vi "Main Page.vi"(8 "error in (no error)":errorcluster, 11 "Node Ptr":T3 format="%.0x") -> (0 "error out":errorcluster)   [LabVIEW 2025, in "Protection and Counter Addon System Explorer.lvlib"]
uses:
  Protection and Counter Addon System Explorer.lvlib
  <vilib>/NI VeriStand/Custom Device API/Custom Device Item Ref.ctl
  SubModules/Frame-Protection-Support/Source/Shared/Types/Protection Type.ctl
  <vilib>/NI/NI VeriStand Hardware Resource Discovery/_Types/Filter Type.ctl
  Addon Shared/Types/986x.ctl
  Addon Shared/SubVIs/GUID Lookup.vi
  <vilib>/NI VeriStand/Custom Device API/NI VeriStand - Get Item Property.vi
  <vilib>/NI VeriStand/Custom Device API/Get Item Property (Boolean).vi
  <vilib>/NI VeriStand/Custom Device API/Get Item Property (String).vi
  <vilib>/NI VeriStand/Custom Device API/Get Item Property (Dependent File).vi
  <vilib>/NI VeriStand/Custom Device API/Custom Device API.lvlib
  <vilib>/NI/NI VeriStand Hardware Resource Discovery/NIVS Hardware Discovery.lvlib
  Addon Shared/Protection and Counter Addon Shared.lvlib
  SubModules/Frame-Protection-Support/Source/Shared/Protection and Counter Support Shared.lvlib
panel:
  in  "Header":cluster{"Section Name":string}={"Section Name"="Addon Settings"}
  in  "Tab Control":T1(tab)
  in  "FD ISO Mode":u32(ring) items=["ISO", "Non ISO", "ISO Legacy"]
  in  "Description":string
  in  "Name":string
  out "Version":string
  in  "Port":string
  in  "CAN Browse":bool
  out "XNET Database":refnum<k21>
  out "XNET Cluster":refnum<k21>
  out "I/O Mode":u32(ring) items=["CAN 2.0", "CAN FD", "CAN FD+BRS"]
  in  "Baud Rate":u64
  in  "Termination":enum16{"Off", "On"}(ring)
  in  "FD Baud Rate":u64
  in  "Use Legacy":bool
  in  "Loop Priority":i32=100 format="%.0p"
  in  "Enable Bitfile":bool
  in  "Bitfile Path":path
  in  "RIO Device":string
  in  "RIO Browse":bool
  in  "Include All Channels":bool
  in  "Default Protect Type":T2
  in  "Default Max Counter Value":dbl
  in  "SHDocVw.IWebBrowser2":refnum<k7>(container)
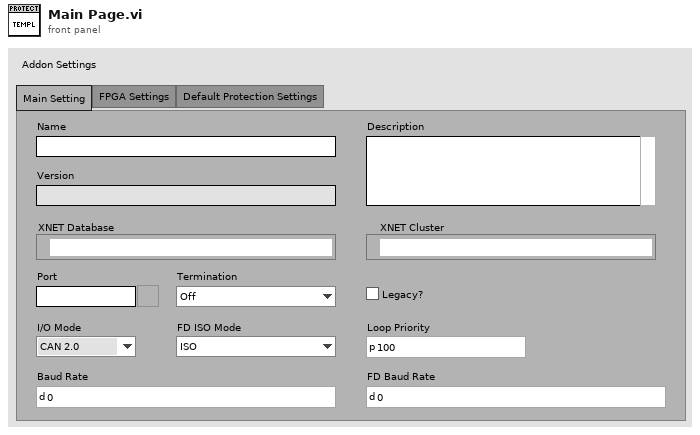
[diagram p1: front panel]
types:
  T1 = enum32{"Main Setting", "FPGA Settings", "Default Protection Settings"}
  T2 = typedef "Protection and Counter Support Shared.lvlib/Protection Type.ctl" = enum16{"Arb ID + Bytes Checksum with Inversion", "Arb ID + Bytes CRC with Inversion", "Reversed Raw Signal Checksum with Inversion", "Concatenated Two's Compliment"}
  T3 = typedef "Custom Device API.lvlib/Custom Device Item Ref.ctl" = u64
  T4 = typedef "Protection and Counter Addon Shared.lvlib/986x.ctl" = cluster{"Enable":bool, "RIO Device":string, "Bitfile":path}
  T5 = typedef "Protection and Counter Addon Shared.lvlib/XNET Settings.ctl" = cluster{"Database":refnum<k21>, "Cluster":refnum<k21>, "Port":string, "Baud rate [Bd]":u64, "Termination":u32, "CAN I/O Mode":u32, "FD Baud rate [Bd]":u64, "Priority":i32, "Use Legacy":bool, "FD ISO Mode":u32, "Default Max Counter Value":dbl, "Default Protect Type":T2, "Include All Channels":bool}
  T6 = typedef "Custom Device API.lvlib/Custom Device Item Info.ctl" = cluster{"Name":string, "Is Channel":bool, "GUID":string, "Is Waveform":bool}
  T7 = typedef "NIVS Hardware Discovery.lvlib/Filter Type.ctl" = enum16{"Device Category", "Product Name", "Ethernet", "XNET", "VISA", "FPGA", "EtherCAT Master", "DAQmx", "GPIB", "Serial"}
  T8 = typedef "Custom Device API.lvlib/Custom Device Commands.ctl" = enum16{"Default", "Item renamed", "Shutdown", "Dynamic button pressed"}
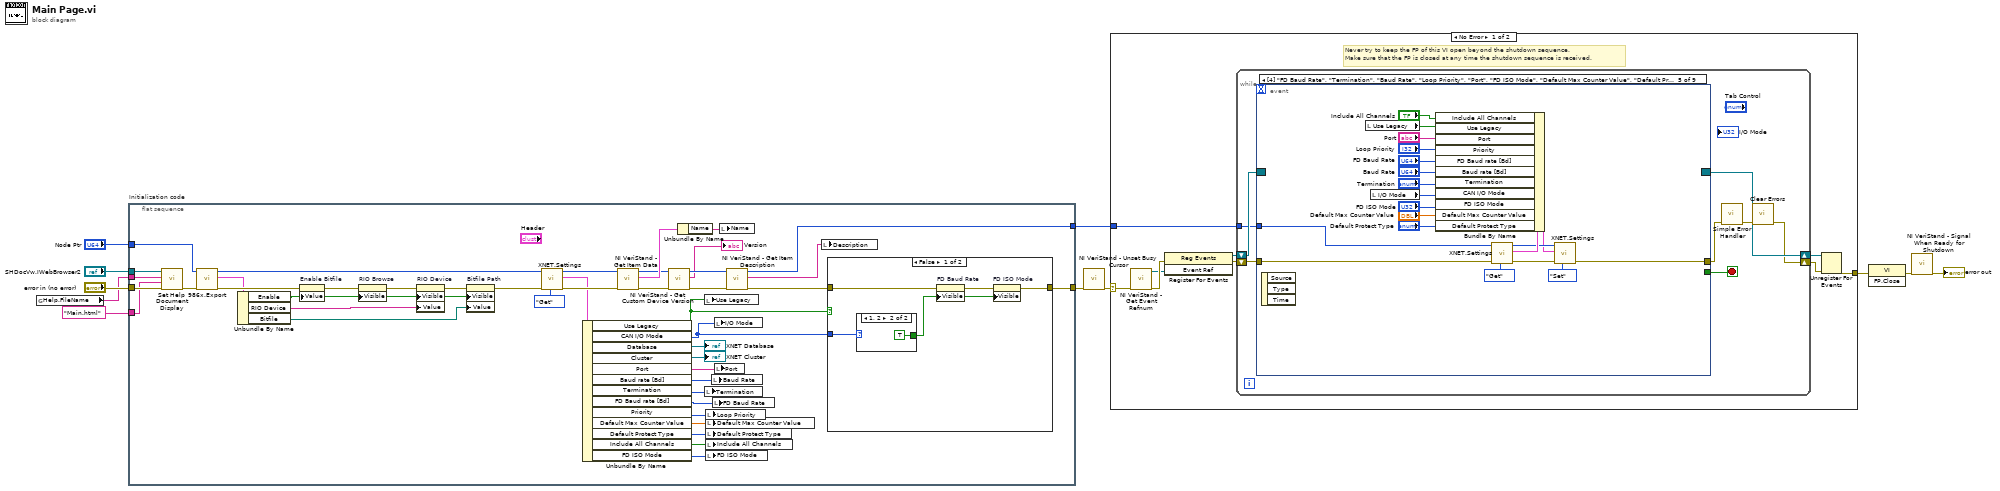
[diagram p0: block diagram]
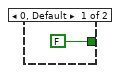
[diagram p2: hidden frame]
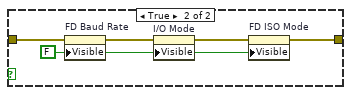
[diagram p3: hidden frame]
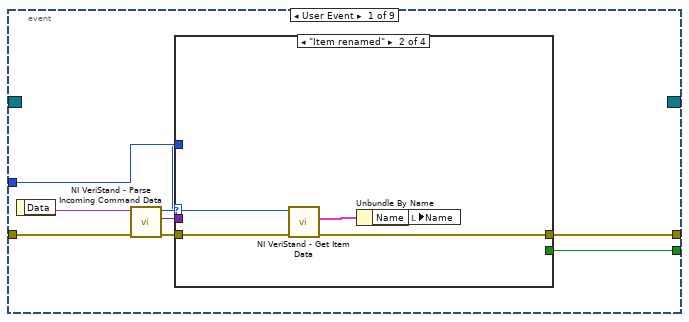
[diagram p4: hidden frame]
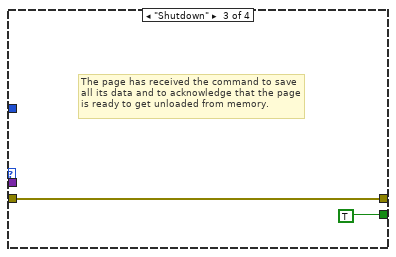
[diagram p6: hidden frame]
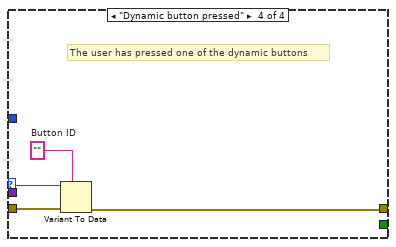
[diagram p7: hidden frame]
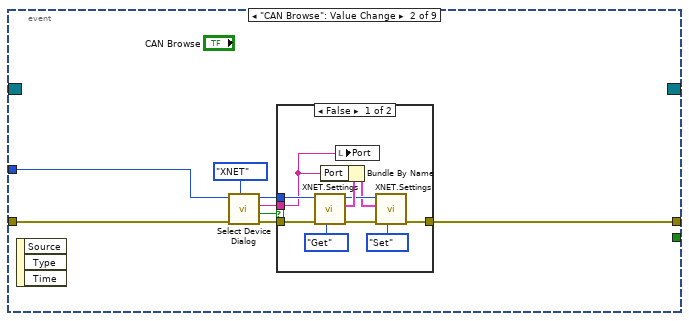
[diagram p8: hidden frame]
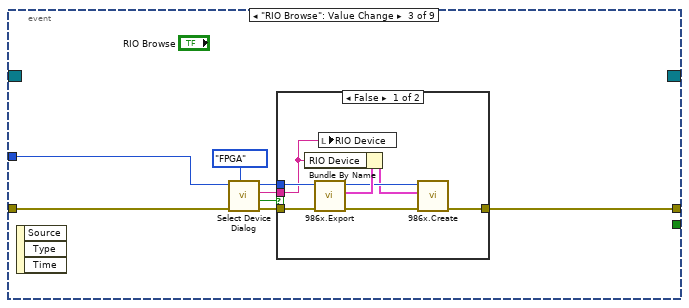
[diagram p10: hidden frame]
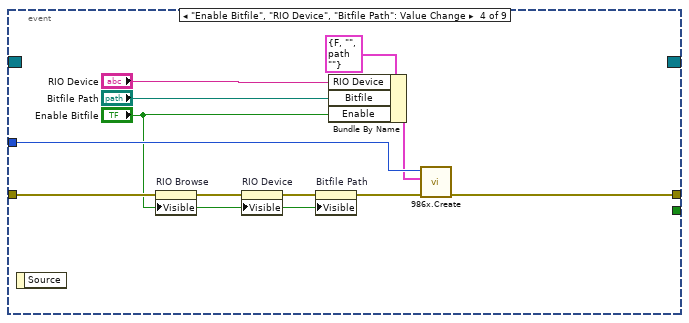
[diagram p12: hidden frame]
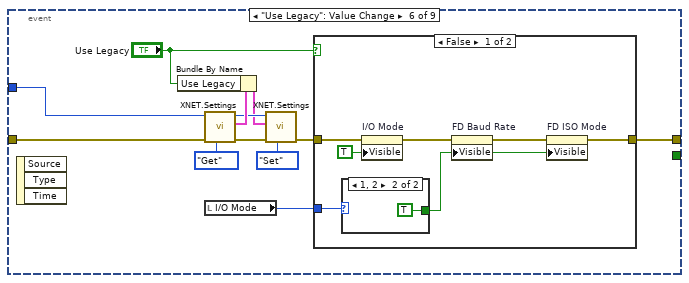
[diagram p13: hidden frame]
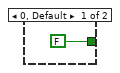
[diagram p14: hidden frame]
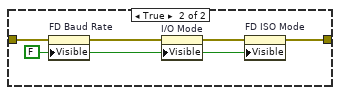
[diagram p15: hidden frame]
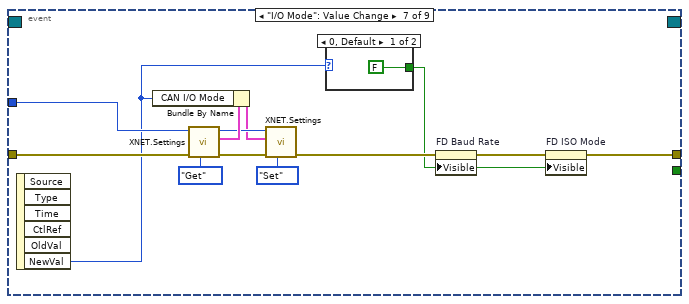
[diagram p16: hidden frame]
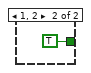
[diagram p17: hidden frame]
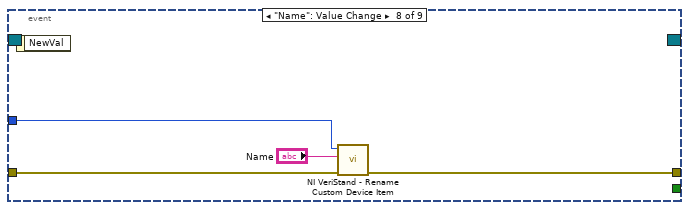
[diagram p18: hidden frame]
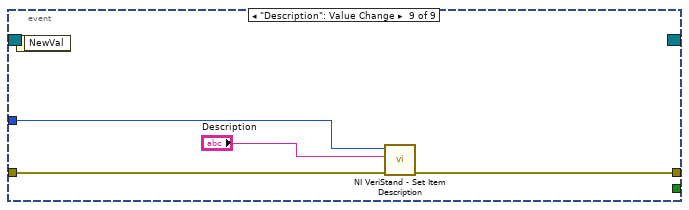
[diagram p19: hidden frame]
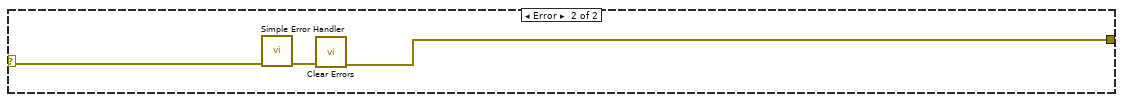
[diagram p20: hidden frame]
diagram:
  n1 = global read "GUID Lookup.vi" "Help.FileName"() -> (w1:string)
  n2 = flat-sequence "Initialization code" {
    tunnel: "error in (no error)" -> [w53]
    tunnel: "Node Ptr" -> [w34]
    tunnel: [w37] -> w7
    tunnel: [w19] -> w4
    tunnel: "SHDocVw.IWebBrowser2" -> [w52]
    tunnel: w1 -> [w51]
    tunnel: "Main.html" ("HTML File") -> [w50]
    frame #0 {
      n3 = call "Set Help Document Display.vi"("error in (no error)"=w53, "HTML File"=w50, "Main CHM File"=w51, "SHDocVw.IWebBrowser2"=w52) -> ("error out"=w35:errorcluster)  [unwired: 7 in]
      n4 = call "986x.Export.vi"("error in (no error)"=w35, "Device Item Ref in"=w34) -> ("error out"=w29:errorcluster, "986x Support"=w27:T4, "Item Ref out"=w33:T3)  [unwired: 7 in]
      n5 = Unbundle By Name(w27) -> ("Enable"=w26:bool, "RIO Device"=w25:string, "Bitfile"=w24:path)
      n6 = property on="Enable Bitfile" class="Bool (strict)"(error in=w29, "Value"=w26) -> (error out=w32:errorcluster)  [unwired: 1 in, 1 out]
      n7 = property on="RIO Browse" class="Bool"(error in=w32, "Visible"=w26) -> (error out=w31:errorcluster)  [unwired: 1 in, 1 out]
      n8 = property on="RIO Device" class="Str"(error in=w31, "Visible"=w26, "Value"=w25) -> (error out=w30:errorcluster)  [unwired: 1 in, 1 out]
      n9 = property on="Bitfile Path" class="Path"(error in=w30, "Visible"=w26, "Value"=w24) -> (error out=w28:errorcluster)  [unwired: 1 in, 1 out]
      n10 = call "XNET.Settings.vi"("Action"=enum8{"Get", "Set"}."Get", "error in (no error)"=w28, "Parent Ref in"=w33) -> ("error out"=w49:errorcluster, "XNET Settings"=w46:T5, "Item Ref out"=w48:T3)  [unwired: 6 in]
      n11 = Unbundle By Name(w46) -> ("Use Legacy"=w38:bool, "CAN I/O Mode"=w36:u32, "Database"=→"XNET Database":refnum<k21>, "Cluster"=→"XNET Cluster":refnum<k21>, "Port"=w43:string, "Baud rate [Bd]"=w42:u64, "Termination"=w41:u32, "FD Baud rate [Bd]"=w40:u64, "Priority"=w39:i32, "Default Max Counter Value"=w15:dbl, "Default Protect Type"=w14:T2, "Include All Channels"=w13:bool, "FD ISO Mode"=w12:u32)
      n12 = call <vilib>:"NI VeriStand - Get Item Data.vi"("error in (no error)"=w49, "Item Ref in"=w48) -> ("error out"=w23:errorcluster, "Item Info"=w55:T6, "Item Ref out"=w22:T3)  [unwired: 7 out]
      n13 = call <vilib>:"NI VeriStand - Get Custom Device Version.vi"("error in (no error)"=w23, "Device Ref in"=w22) -> ("error out"=w18:errorcluster, "Value"=→"Version":string, "Device Ref out"=w21:T3)  [unwired: 7 in]
      n14 = Unbundle By Name(w55) -> ("Name"=w54:string)
      n15 = local write "Use Legacy"(w38) -> ()
      n16 = local write "Termination"(w41) -> ()
      n17 = local write "Loop Priority"(w39) -> ()
      n18 = local write "Default Max Counter Value"(w15) -> ()
      n19 = local write "Default Protect Type"(w14) -> ()
      n20 = local write "Include All Channels"(w13) -> ()
      n21 = local write "FD ISO Mode"(w12) -> ()
      n22 = local write "Baud Rate"(w42) -> ()
      n23 = local write "FD Baud Rate"(w40) -> ()
      n24 = local write "I/O Mode"(w36) -> ()
      n25 = local write "Port"(w43) -> ()
      n26 = local write "Name"(w54) -> ()
      n27 = call <vilib>:"NI VeriStand - Get Item Description.vi"("error in (no error)"=w18, "Item Ref in"=w21) -> ("error out"=w17:errorcluster, "Description"=w16:string, "Item Ref out"=w19:T3)  [unwired: 6 in, 1 out]
      n28 = local write "Description"(w16) -> ()
      n29 = case shown="False" w38 {
        tunnel: w17 -> [w59 w66]
        tunnel: [w57 w64] -> w37
        tunnel: w36 -> [w60 _]
        frame False {
          n30 = case shown="1, 2" w60 {
            tunnel: [FALSE TRUE] -> w56
            frame 0, Default {
            }
            frame 1, 2 {
            }
          }
          n31 = property on="FD Baud Rate" class="DigNum (strict)"(error in=w59, "Visible"=w56) -> (error out=w58:errorcluster)  [unwired: 1 in, 1 out]
          n32 = property on="FD ISO Mode" class="Ring (strict)"(error in=w58, "Visible"=w56) -> (error out=w57:errorcluster)  [unwired: 1 in, 1 out]
        }
        frame True {
          w63 = FALSE ("Visible")
          n33 = property on="FD Baud Rate" class="DigNum (strict)"(error in=w66, "Visible"=w63) -> (error out=w67:errorcluster)  [unwired: 1 in, 1 out]
          n34 = property on="I/O Mode" class="Ring (strict)"(error in=w67, "Visible"=w63) -> (error out=w65:errorcluster)  [unwired: 1 in, 1 out]
          n35 = property on="FD ISO Mode" class="Ring (strict)"(error in=w65, "Visible"=w63) -> (error out=w64:errorcluster)  [unwired: 1 in, 1 out]
        }
      }
    }
  }
  n36 = call <vilib>:"NI VeriStand - Unset Busy Cursor.vi"("error in (no error)"=w7) -> ("error out"=w6:errorcluster)  [unwired: 10 out]
  n37 = case shown="No Error" w6 {
    selector: w6 -> [w68 w223]
    tunnel: [w73 w221] -> w11
    tunnel: w4 -> [w69 _]
    frame No Error {
      # "Never try to keep the FP of this VI open beyond the shutdown sequence.\nMake sure that the FP is closed at any time the shutdown sequence is received."
      n38 = call <vilib>:"NI VeriStand - Get Event Refnum.vi"("error in (no error)"=w68) -> ("error out"=w76:errorcluster, "Event Ref"=w72:refnum<user-event>)  [unwired: 9 out]
      n39 = register-events(error in=w76, w72) -> (reference out=w70:refnum<event-registration>, error out=w71:errorcluster)  [unwired: 1 in]
      n40 = while {
        tunnel: w69 -> [w80]
        shift-right: [w77] -> w74
        shift-left: w71 -> [w83]
        shift-right: [w84] -> w75
        shift-left: w70 -> [w82]
        stop <- w81 stop-if-true
        n41 = event shown="[4] \"FD Baud Rate\", \"Termination\", \"Baud Rate\", \"Loop Priority\", \"Port\", \"FD ISO Mode\", \"Default Max Counter Value\", \"Default Protect Type\", \"Include All Channels\": Value Change" {
          selector: w82 -> [_ _ _ _ _ _ _ _ _]
          dyn-events: [_ _ _ _ _ _ _ _ _] -> w84
          timeout: _ -> [_ _ _ _ _ _ _ _ _]
          tunnel: w83 -> [w92 w107 w126 w148 w165 w177 w204 w216 w220]
          tunnel: [w88 _ _ _ _ _ _ _ _] -> w81
          tunnel: [w87 w105 w124 w151 w164 w173 w199 w215 w219] -> w79
          tunnel: w80 -> [w86 w106 w125 w146 w163 w176 w203 w214 w218]
          event User Event {
            n42 = event-data() -> ("Data"=w91:string)  [unwired: 1 out]
            n43 = call <vilib>:"NI VeriStand - Parse Incoming Command Data.vi"("error in (no error)"=w92, "Incoming data"=w91) -> ("error out"=w90:errorcluster, "Outgoing data"=w85:variant, "Action"=w89:T8)  [unwired: 7 out]
            n44 = case shown="\"Item renamed\"" w89 {
              tunnel: w90 -> [w93 w98 w99 w104]
              tunnel: [_ _ TRUE _] -> w88
              tunnel: [w93 w95 w99 w101] -> w87
              tunnel: w86 -> [_ w97 _ _]
              tunnel: w85 -> [_ _ _ w103]
              frame "Default", Default {
              }
              frame "Item renamed" {
                n45 = call <vilib>:"NI VeriStand - Get Item Data.vi"("error in (no error)"=w98, "Item Ref in"=w97) -> ("error out"=w95:errorcluster, "Item Info"=w96:T6)  [unwired: 8 out]
                n46 = Unbundle By Name(w96) -> ("Name"=w94:string)
                n47 = local write "Name"(w94) -> ()
              }
              frame "Shutdown" {
                # "The page has received the command to save all its data and to acknowledge that the page is ready to get unloaded from memory."
              }
              frame "Dynamic button pressed" {
                w102 = ""  # Button ID
                # "The user has pressed one of the dynamic buttons"
                n48 = Variant To Data(error in=w104, type=w102, Variant=w103) -> (error out=w101:errorcluster)  [unwired: 1 out]
              }
            }
          }
          event "CAN Browse": Value Change {
            n49 = event-data() -> ()  [unwired: 4 out]
            n50 = call <vilib>:"Select Device Dialog.vi"("Filter Type"=Filter_Type."XNET", "error in (no error)"=w107, "Item Ref in"=w106) -> ("error out"=w111:errorcluster, "Cancelled?"=w110:bool, "Selected Alias"=w109:string, "Item Ref out"=w112:T3)  [unwired: 5 in]
            n51 = case shown="False" w110 {
              tunnel: w112 -> [w120 _]
              tunnel: [w117 w123] -> w105
              tunnel: w111 -> [w114 w123]
              tunnel: w109 -> [w113 _]
              frame False {
                n52 = call "XNET.Settings.vi"("Action"=enum8{"Get", "Set"}."Get", "error in (no error)"=w114, "Parent Ref in"=w120) -> ("error out"=w115:errorcluster, "XNET Settings"=w121:T5, "Item Ref out"=w118:T3)  [unwired: 6 in]
                n53 = Bundle By Name(cluster=w121, "Port"=w113) -> (w116:T5)
                n54 = local write "Port"(w113) -> ()
                n55 = call "XNET.Settings.vi"("Action"=enum8{"Get", "Set"}."Set", "error in (no error)"=w115, "XNET Settings"=w116, "Parent Ref in"=w118) -> ("error out"=w117:errorcluster)  [unwired: 5 in, 2 out]
              }
              frame True {
              }
            }
          }
          event "RIO Browse": Value Change {
            n56 = event-data() -> ()  [unwired: 4 out]
            n57 = call <vilib>:"Select Device Dialog.vi"("Filter Type"=Filter_Type."FPGA", "error in (no error)"=w126, "Item Ref in"=w125) -> ("error out"=w130:errorcluster, "Cancelled?"=w129:bool, "Selected Alias"=w128:string, "Item Ref out"=w131:T3)  [unwired: 5 in]
            n58 = case shown="False" w129 {
              tunnel: w131 -> [w138 _]
              tunnel: [w133 w140] -> w124
              tunnel: w130 -> [w137 w140]
              tunnel: w128 -> [w136 _]
              frame False {
                n59 = call "986x.Export.vi"("error in (no error)"=w137, "Device Item Ref in"=w138) -> ("error out"=w135:errorcluster, "986x Support"=w139:T4, "Item Ref out"=w134:T3)  [unwired: 7 in]
                n60 = Bundle By Name(cluster=w139, "RIO Device"=w136) -> (w132:T4)
                n61 = local write "RIO Device"(w136) -> ()
                n62 = call "986x.Create.vi"("error in (no error)"=w135, "986x Support"=w132, "Device Item Ref in"=w134) -> ("error out"=w133:errorcluster)  [unwired: 7 in, 1 out]
              }
              frame True {
              }
            }
          }
          event "Enable Bitfile", "RIO Device", "Bitfile Path": Value Change {
            n63 = event-data() -> ()  [unwired: 2 out]
            n64 = property on="RIO Browse" class="Bool"(error in=w148, "Visible"="Enable Bitfile") -> (error out=w149:errorcluster)  [unwired: 1 in, 1 out]
            n65 = property on="RIO Device" class="Str"(error in=w149, "Visible"="Enable Bitfile") -> (error out=w150:errorcluster)  [unwired: 1 in, 1 out]
            n66 = property on="Bitfile Path" class="Path"(error in=w150, "Visible"="Enable Bitfile") -> (error out=w147:errorcluster)  [unwired: 1 in, 1 out]
            n67 = Bundle By Name(cluster=T4 {"Enable"=FALSE, "RIO Device"="", "Bitfile"=path ""} ("986x Support"), "RIO Device"="RIO Device", "Bitfile"="Bitfile Path", "Enable"="Enable Bitfile") -> (w144:T4)
            n68 = call "986x.Create.vi"("error in (no error)"=w147, "986x Support"=w144, "Device Item Ref in"=w146) -> ("error out"=w151:errorcluster)  [unwired: 7 in, 1 out]
          }
          event "FD Baud Rate", "Termination", "Baud Rate", "Loop Priority", "Port", "FD ISO Mode", "Default Max Counter Value", "Include All Channels": Value Change {
            n69 = event-data() -> ()  [unwired: 4 out]
            n70 = local read "Use Legacy"() -> (w157:bool)
            n71 = local read "I/O Mode"() -> (w156:u32)
            n72 = call "XNET.Settings.vi"("Action"=enum8{"Get", "Set"}."Get", "error in (no error)"=w165, "Parent Ref in"=w163) -> ("error out"=w166:errorcluster, "XNET Settings"=w170:T5, "Item Ref out"=w168:T3)  [unwired: 6 in]
            n73 = Bundle By Name(cluster=w170, "Include All Channels"="Include All Channels", "Use Legacy"=w157, "Port"="Port", "Priority"="Loop Priority", "FD Baud rate [Bd]"="FD Baud Rate", "Baud rate [Bd]"="Baud Rate", "Termination"="Termination", "CAN I/O Mode"=w156, "FD ISO Mode"="FD ISO Mode", "Default Max Counter Value"="Default Max Counter Value", "Default Protect Type"="Default Protect Type") -> (w167:T5)
            n74 = call "XNET.Settings.vi"("Action"=enum8{"Get", "Set"}."Set", "error in (no error)"=w166, "XNET Settings"=w167, "Parent Ref in"=w168) -> ("error out"=w164:errorcluster)  [unwired: 5 in, 2 out]
          }
          event "Use Legacy": Value Change {
            n75 = event-data() -> ()  [unwired: 4 out]
            n76 = call "XNET.Settings.vi"("Action"=enum8{"Get", "Set"}."Get", "error in (no error)"=w177, "Parent Ref in"=w176) -> ("error out"=w178:errorcluster, "XNET Settings"=w182:T5, "Item Ref out"=w180:T3)  [unwired: 6 in]
            n77 = Bundle By Name(cluster=w182, "Use Legacy"="Use Legacy") -> (w179:T5)
            n78 = local read "I/O Mode"() -> (w172:u32)
            n79 = call "XNET.Settings.vi"("Action"=enum8{"Get", "Set"}."Set", "error in (no error)"=w178, "XNET Settings"=w179, "Parent Ref in"=w180) -> ("error out"=w174:errorcluster)  [unwired: 5 in, 2 out]
            n80 = case shown="False" "Use Legacy" {
              tunnel: w174 -> [w189 w196]
              tunnel: [w185 w194] -> w173
              tunnel: w172 -> [w190 _]
              frame False {
                n81 = case shown="1, 2" w190 {
                  tunnel: [FALSE TRUE] -> w184
                  frame 0, Default {
                  }
                  frame 1, 2 {
                  }
                }
                n82 = property on="I/O Mode" class="Ring (strict)"(error in=w189, "Visible"=TRUE) -> (error out=w188:errorcluster)  [unwired: 1 in, 1 out]
                n83 = property on="FD Baud Rate" class="DigNum (strict)"(error in=w188, "Visible"=w184) -> (error out=w186:errorcluster)  [unwired: 1 in, 1 out]
                n84 = property on="FD ISO Mode" class="Ring (strict)"(error in=w186, "Visible"=w184) -> (error out=w185:errorcluster)  [unwired: 1 in, 1 out]
              }
              frame True {
                w193 = FALSE ("Visible")
                n85 = property on="FD Baud Rate" class="DigNum (strict)"(error in=w196, "Visible"=w193) -> (error out=w197:errorcluster)  [unwired: 1 in, 1 out]
                n86 = property on="I/O Mode" class="Ring (strict)"(error in=w197, "Visible"=w193) -> (error out=w195:errorcluster)  [unwired: 1 in, 1 out]
                n87 = property on="FD ISO Mode" class="Ring (strict)"(error in=w195, "Visible"=w193) -> (error out=w194:errorcluster)  [unwired: 1 in, 1 out]
              }
            }
          }
          event "I/O Mode": Value Change {
            n88 = event-data() -> ("NewVal"=w201:u32)  [unwired: 6 out]
            n89 = call "XNET.Settings.vi"("Action"=enum8{"Get", "Set"}."Get", "error in (no error)"=w204, "Parent Ref in"=w203) -> ("error out"=w205:errorcluster, "XNET Settings"=w209:T5, "Item Ref out"=w207:T3)  [unwired: 6 in]
            n90 = Bundle By Name(cluster=w209, "CAN I/O Mode"=w201) -> (w206:T5)
            n91 = call "XNET.Settings.vi"("Action"=enum8{"Get", "Set"}."Set", "error in (no error)"=w205, "XNET Settings"=w206, "Parent Ref in"=w207) -> ("error out"=w202:errorcluster)  [unwired: 5 in, 2 out]
            n92 = case shown="0, Default" w201 {
              tunnel: [FALSE TRUE] -> w198
              frame 0, Default {
              }
              frame 1, 2 {
              }
            }
            n93 = property on="FD Baud Rate" class="DigNum (strict)"(error in=w202, "Visible"=w198) -> (error out=w200:errorcluster)  [unwired: 1 in, 1 out]
            n94 = property on="FD ISO Mode" class="Ring (strict)"(error in=w200, "Visible"=w198) -> (error out=w199:errorcluster)  [unwired: 1 in, 1 out]
          }
          event "Name": Value Change {
            n95 = event-data() -> ()  [unwired: 2 out]
            n96 = call <vilib>:"NI VeriStand - Rename Custom Device Item.vi"("error in (no error)"=w216, "New Name"="Name", "Item Ref in"=w214) -> ("error out"=w215:errorcluster)  [unwired: 1 in, 7 out]
          }
          event "Description": Value Change {
            n97 = event-data() -> ()  [unwired: 2 out]
            n98 = call <vilib>:"NI VeriStand - Set Item Description.vi"("error in (no error)"=w220, "Description"="Description", "Item Ref in"=w218) -> ("error out"=w219:errorcluster)  [unwired: 6 in, 2 out]
          }
        }
        n99 = call <vilib>:"Simple Error Handler.vi"("error in (no error)"=w79) -> ("error out"=w78:errorcluster)  [unwired: 1 in, 7 out]
        n100 = call <vilib>:"Clear Errors.vi"("error in (no error)"=w78) -> ("error out"=w77:errorcluster)  [unwired: 1 in, 5 out]
      }
      n101 = Unregister For Events(event registration refnum=w75, error in=w74) -> (error out=w73:errorcluster)
    }
    frame Error {
      n102 = call <vilib>:"Simple Error Handler.vi"("error in (no error)"=w223) -> ("error out"=w222:errorcluster)  [unwired: 1 in, 7 out]
      n103 = call <vilib>:"Clear Errors.vi"("error in (no error)"=w222) -> ("error out"=w221:errorcluster)  [unwired: 1 in, 5 out]
    }
  }
  n104 = invoke class="VI" method="FP.Close"(error in=w11) -> (error out=w10:errorcluster)  [unwired: 2 in, 2 out]
  n105 = call <vilib>:"NI VeriStand - Signal When Ready for Shutdown.vi"("error in (no error)"=w10) -> ("error out"=→"error out":errorcluster)  [unwired: 10 out]
